vi "check IDN Query Value.vi"(8 "error in (no error)":errorcluster, 11 "LTE in":refnum<class "LTE.lvclass">) -> (0 "error out":errorcluster, 2 "Connected":bool, 3 "LTE out":refnum<class "LTE.lvclass">)   [LabVIEW 2023, in "ANRITSU Call Box.lvlib" / "LTE.lvclass"]
uses:
  LTE.lvclass
  LTE.lvclass/LTE.ctl
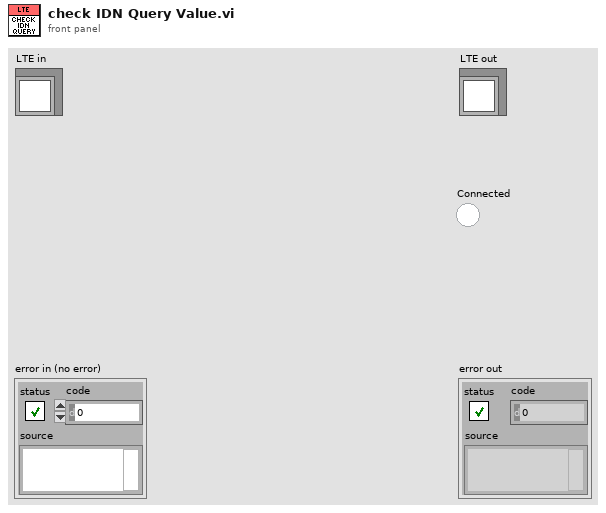
[diagram p1: front panel]
types:
  T1 = typedef "ANRITSU Call Box.lvlib/Call Device - Protocol Type Selector.ctl" = enum16{"8000A - NR", "8000A - LTE", "882xC - LTE"}
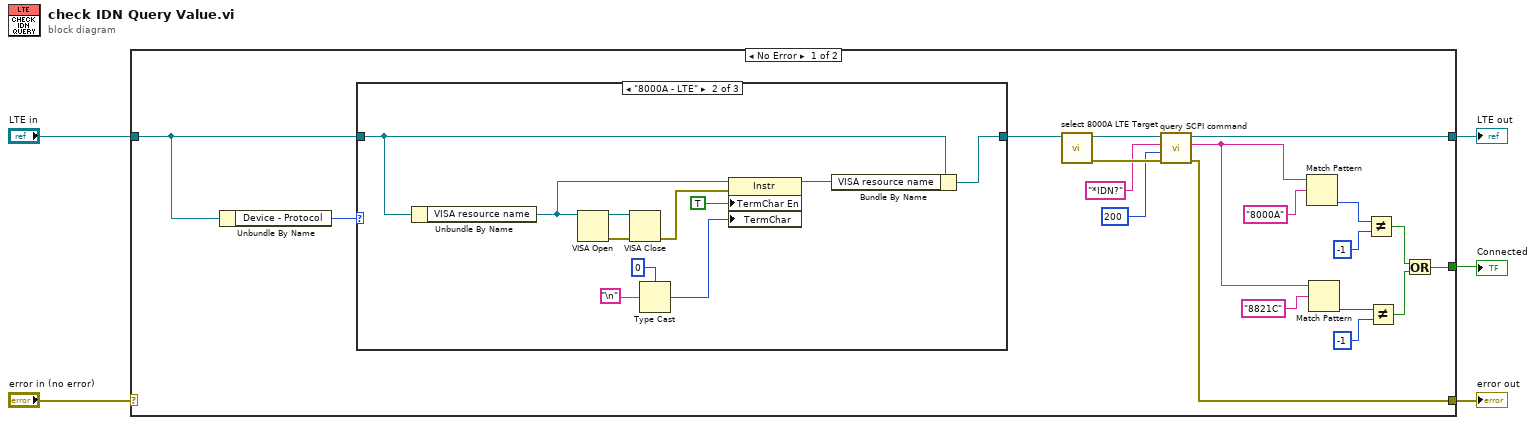
[diagram p0: block diagram]
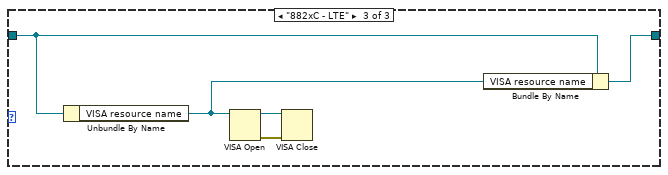
[diagram p3: hidden frame]
diagram:
  n1 = case shown="No Error" "error in (no error)" {
    selector: "error in (no error)" -> [_ w43]
    tunnel: [w14 w43] -> w4
    tunnel: [w21 w42] -> w2
    tunnel: "LTE in" -> [w24 w42]
    tunnel: [w8 _] -> w1
    frame No Error {
      n2 = Unbundle By Name(w24) -> ("Device - Protocol"=w13:T1)
      n3 = case shown="\"8000A - LTE\"" w13 {
        tunnel: w24 -> [w25 w28 w38]
        tunnel: [w25 w26 w37] -> w23
        frame "8000A - NR", Default {
        }
        frame "8000A - LTE" {
          n4 = Unbundle By Name(w28) -> ("VISA resource name"=w35:refnum<visa-resource-name>)
          n5 = VISA Open(VISA resource name=w35) -> (VISA resource name=w29:refnum<visa-resource-name>, error out=w36:errorcluster)  [unwired: 4 in]
          n6 = VISA Close(VISA resource name=w29, error in (no error)=w36) -> (error out=w34:errorcluster)
          n7 = Type Cast(type=u8 0 ("Message Based Settings:Termination Character"), x="\n") -> (*(type *) &x=w30:u8)
          n8 = property class="Instr"(reference=w35, error in=w34, "TermChar En"=TRUE ("Message Based Settings:Termination Character Enable"), "TermChar"=w30) -> (reference out=w27:refnum<visa-resource-name>)  [unwired: 1 out]
          n9 = Bundle By Name(cluster=w28, "VISA resource name"=w27) -> (w26:refnum<class "LTE.lvclass">)
        }
        frame "882xC - LTE" {
          n10 = Unbundle By Name(w38) -> ("VISA resource name"=w40:refnum<visa-resource-name>)
          n11 = VISA Open(VISA resource name=w40) -> (VISA resource name=w39:refnum<visa-resource-name>, error out=w41:errorcluster)  [unwired: 4 in]
          n12 = VISA Close(VISA resource name=w39, error in (no error)=w41) -> ()  [unwired: 1 out]
          n13 = Bundle By Name(cluster=w38, "VISA resource name"=w40) -> (w37:refnum<class "LTE.lvclass">)
        }
      }
      n14 = call "select 8000A LTE Target.vi"("LTE in"=w23) -> ("error out"=w20:errorcluster, "LTE out"=w22:refnum<class "LTE.lvclass">)  [unwired: 9 in]
      n15 = call "query SCPI command.vi"("error in (no error)"=w20, "Read Buffer Length"=u32 200, "SCPI Command"="*IDN?" ("write buffer"), "LTE in"=w22) -> ("error out"=w14:errorcluster, "Read Buffer String"=w12:string, "LTE out"=w21:refnum<class "LTE.lvclass">)  [unwired: 5 in]
      n16 = Match Pattern(string=w12, regular expression="8000A") -> (offset past match=w16:i32)  [unwired: 1 in, 3 out]
      n17 = Match Pattern(string=w12, regular expression="8821C") -> (offset past match=w10:i32)  [unwired: 1 in, 3 out]
      n18 = Not Equal?(x=w16, y=-1) -> (x != y?=w7:bool)
      n19 = Not Equal?(x=w10, y=-1) -> (x != y?=w6:bool)
      n20 = Or(x=w7, y=w6) -> (x .or. y?=w8:bool)
    }
    frame Error {
    }
  }
  "error out" <- w4
  "LTE out" <- w2
  "Connected" <- w1
